vi "FilterComparison.vi"() -> ()   [LabVIEW 2019]
uses:
  <vilib>/Rock Robotics/WPI/ThirdParty/JAS_Junk/TrajLib/Trajectory_Library.lvlib
  <vilib>/Rock Robotics/WPI/ThirdParty/JAS_Junk/TrajLib/LinearFilter_MovingAvg_Execute.vi
  <vilib>/Rock Robotics/WPI/ThirdParty/JAS_Junk/TrajLib/LinearFilter_LP_BW1_Execute.vi
  <vilib>/Rock Robotics/WPI/ThirdParty/JAS_Junk/TrajLib/LinearFilter_LP_BW2_Execute.vi
  <vilib>/Rock Robotics/WPI/ThirdParty/JAS_Junk/TrajLib/LinearFilter_HP_BW1_Execute.vi
  <vilib>/Rock Robotics/WPI/ThirdParty/JAS_Junk/TrajLib/LinearFilter_HP_BW2_Execute.vi
panel:
  out "Wait Adjust":dbl format="%11.3f"
  in  "Auto / Manual":bool=TRUE
  in  "Enable\nNoise":bool=TRUE
  in  "Filter Enable":bool=TRUE
  in  "Use White Noise":bool=TRUE
  in  "Tab Control 2":T1(tab)
  out "Avg3":cluster{dbl, dbl, "Value_Output":dbl}(graph)
  out "Avg3 Out Dial":dbl(knob)=-2.895988890827539e-05 scale=-20.0..20.0
  out "Avg3 Out":dbl format="%11.3f"
  out "Med3":cluster{dbl, dbl, "Value_Output":dbl}(graph)
  out "Med3 Out":dbl format="%11.3f"
  out "Med3 Out Dial":dbl(knob)=-2.895988890827539e-05 scale=-20.0..20.0
  out "Avg7":cluster{dbl, dbl, "Value_Output":dbl}(graph)
  out "Avg7 Out":dbl format="%11.3f"
  out "Avg7 Out Dial":dbl(knob)=-2.895988890827539e-05 scale=-20.0..20.0
  out "Med7":cluster{dbl, dbl, "Value_Output":dbl}(graph)
  out "Med7 Out":dbl format="%11.3f"
  out "Med7 Out Dial":dbl(knob)=-2.895988890827539e-05 scale=-20.0..20.0
  out "LP BW 2":cluster{dbl, dbl, "Output_Value":dbl}(graph)
  out "LP BW 1 Out":dbl format="%11.3f"
  out "Low Pass 1st order Butterworth FIlter":dbl(knob)=-2.895988890827539e-05 scale=-20.0..20.0
  out "Fc 2":dbl format="%11.3f"
  out "LP BW 2":cluster{dbl, dbl, "Output_Value":dbl}(graph)
  out "LP BW 2 Out":dbl format="%11.3f"
  out "Low Pass 2nd order Butterworth Filter":dbl(knob)=-2.895988890827539e-05 scale=-20.0..20.0
  out "Fc 3":dbl format="%11.3f"
  out "HP BW 1":cluster{dbl, dbl, "Output_Value":dbl}(graph)
  out "HP BW 1":dbl format="%11.3f"
  out "High Pass 1st order Butterworth Filter":dbl(knob)=-2.895988890827539e-05 scale=-20.0..20.0
  out "HP  BW 2":cluster{dbl, dbl, "Output_Value":dbl}(graph)
  out "HP BW 2 out":dbl format="%11.3f"
  out "High Pass 2nd order Butterworth Filter":dbl(knob)=-2.895988890827539e-05 scale=-20.0..20.0
  out "Cutoff Freq\nHP BW 2":dbl format="%11.3f"
  out "Duration":dbl format="%11.3f"
  out "Late":dbl format="%11.3f"
  in  "Manual\nInput":dbl(slide) min=-12.0 max=12.0 scale=-12.0..12.0
  out "Raw Noise":dbl(knob)=-2.895988890827539e-05 scale=-20.0..20.0
  out "Raw Noise":dbl format="%11.3f"
  out "Actual Input":dbl(knob)=-2.895988890827539e-05 scale=-20.0..20.0
  out "Actual Input":dbl format="%11.3f"
  in  "Time Const (Sec)":dbl=0.08 min=0.0 step=0.001 format="%10.4f"
  out "Input":cluster{"Manual\nInput":dbl, dbl, "f":dbl}(graph)
  out "Meas Dial":dbl(knob)=-2.895988890827539e-05 scale=-20.0..20.0
  out "Measured Value":dbl format="%11.3f"
  # "Comparison of Different Filters"
  # "Loop Information"
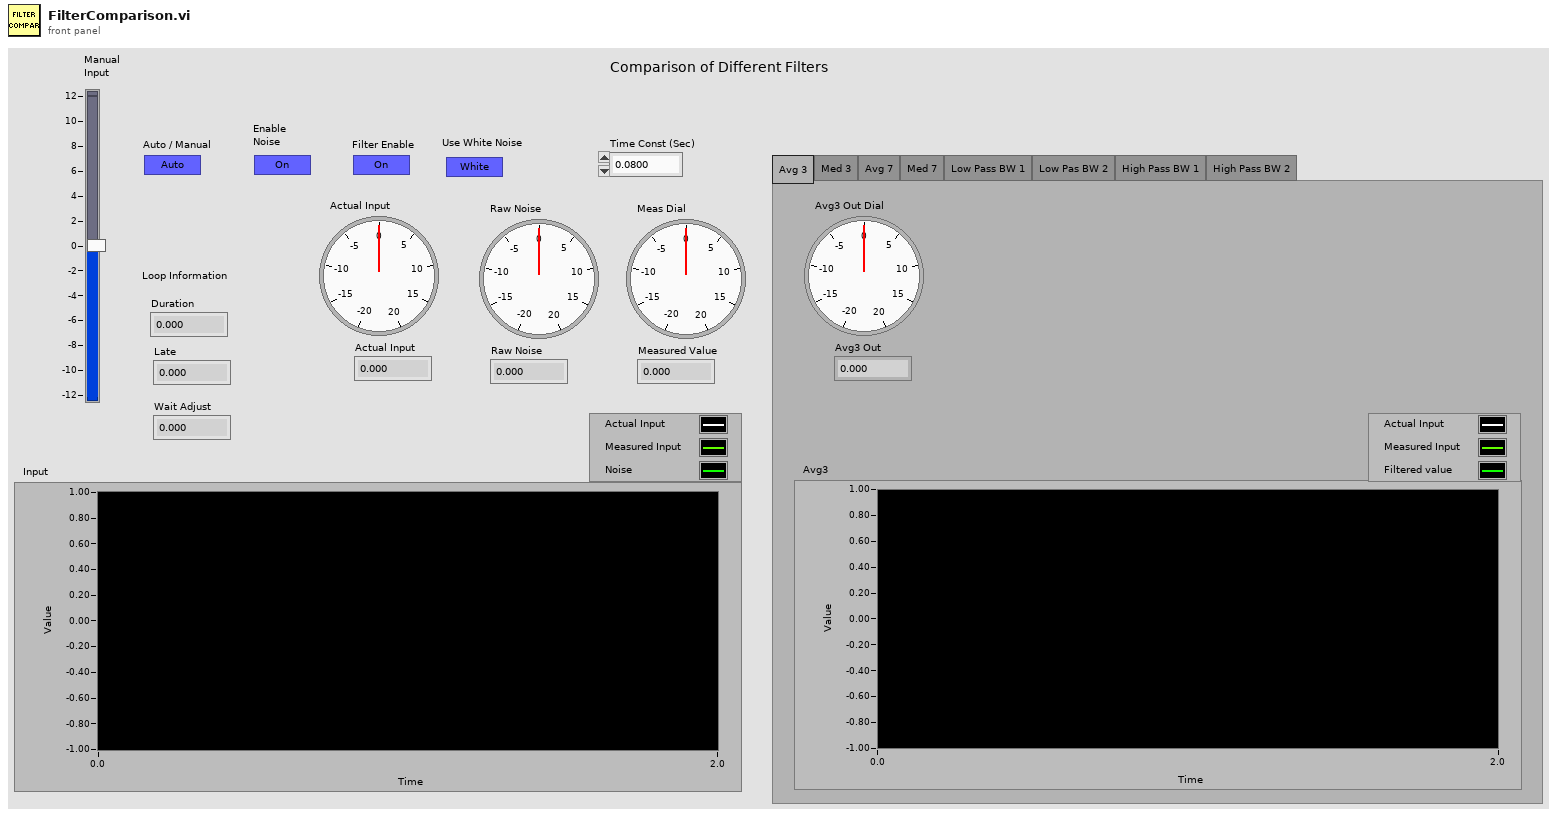
[diagram p1: front panel]
types:
  T1 = enum32{"Avg 3", "Med 3", "Avg 7", "Med 7", "Low Pass BW 1", "Low Pas BW 2", "High Pass BW 1", "High Pass BW 2"}
  T2 = cluster{"Manual\nInput":dbl, dbl, "MedianValue":dbl}
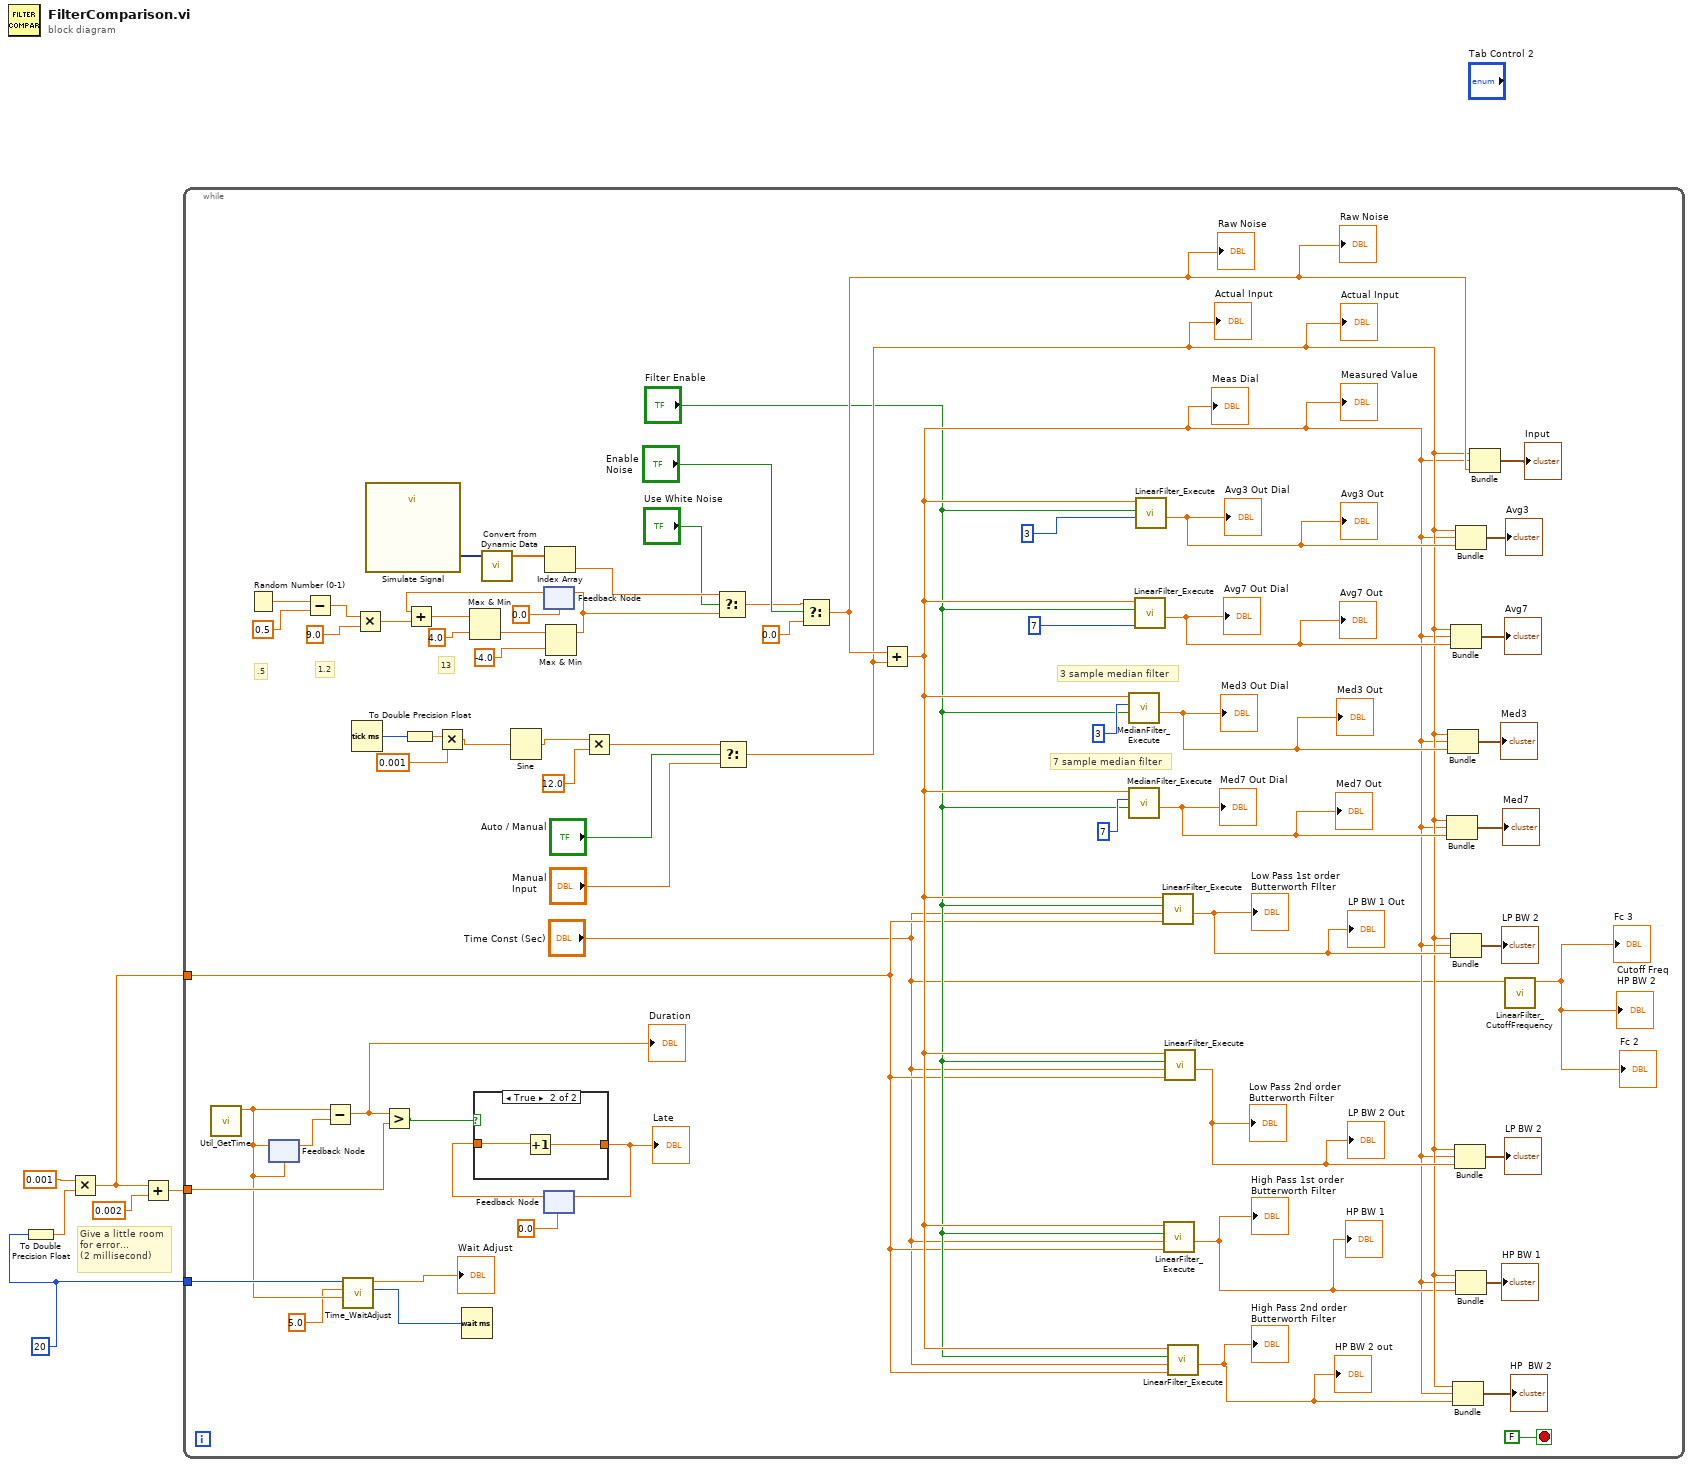
[diagram p0: block diagram]
diagram:
  w4 = u32 20 ("milliseconds to wait")
  # "Give a little room\nfor error...\n(2 millisecond)"
  n1 = To Double Precision Float(number=w4) -> (double precision float=w6:dbl)
  n2 = Multiply(x=0.001, y=w6) -> (x*y=w1:dbl)
  n3 = Add(x=w1, y=0.002) -> (x+y=w3:dbl)
  n4 = while {
    tunnel: w4 -> [w12]
    tunnel: w3 -> [w30]
    tunnel: w1 -> [w14]
    stop <- FALSE stop-if-true
    # "7 sample median filter"
    # "3 sample median filter"
    # "13"
    # "1.2"
    # ".5"
    n5 = call <vilib>:"Util_GetTime.vi"() -> ("FPGA_Time_Seconds"=w11:dbl)  [unwired: 9 in, 2 out]
    n6 = Random Number (0-1)() -> (number: 0 to 1=w70:dbl)
    n7 = feedback-in #1(w11) -> ()
    n8 = feedback #1(w11) -> (w33:dbl)
    n9 = Subtract(x=w70, y=0.5) -> (x-y=w66:dbl)
    n10 = Subtract(x=w11, y=w33) -> (x-y=w31:dbl)
    "Duration" <- w31
    n11 = call <vilib>:"Time_WaitAdjust.vi"("PassthroughTime_SEC"=w11, "MaxAdjustment_MS"=5.0 ("MaxDeviation_MS"), "DesiredLoopTime_MS"=w12) -> ("AdjustedWaitTime_MS"=w9:u32, "Offset_MS"=→"Wait Adjust":dbl)  [unwired: 7 in]
    n12 = Tick Count (ms)() -> (millisecond timer value=w59:u32)
    n13 = Multiply(x=w66, y=9.0) -> (x*y=w65:dbl)
    n14 = call "Simulate Signal"() -> ("DC with Uniform Noise"=w47:dynamicdata)  [unwired: 14 in, 1 out]
    n15 = Greater?(x=w31, y=w30) -> (0:w32:bool)
    n16 = To Double Precision Float(number=w59) -> (double precision float=w60:dbl)
    n17 = Multiply(x=w60, y=0.001) -> (x*y=w57:dbl)
    n18 = Wait (ms)(milliseconds to wait=w9) -> ()  [unwired: 1 out]
    n19 = call "Convert from Dynamic Data"("Dynamic Data Type"=w47) -> ("Array"=w46:dbl[])  [unwired: 3 in]
    n20 = Sine(x=w57) -> (sin(x)=w56:dbl)
    n21 = feedback #2(0.0) -> (w67:dbl)
    n22 = Add(x=w67, y=w65) -> (x+y=w69:dbl)
    n23 = Max & Min(x=w69, y=4.0) -> (min(x,y)=w68:dbl)  [unwired: 1 out]
    n24 = feedback #3(0.0) -> (w40:dbl)
    n25 = case shown="True" w32 {
      tunnel: [w76 w78] -> w41
      tunnel: w40 -> [w76 w77]
      frame False {
      }
      frame True {
        n26 = Increment(x=w77) -> (x+1=w78:dbl)
      }
    }
    "Late" <- w41
    n27 = feedback-in #3(w41) -> ()
    n28 = Index Array(array=w46) -> (element=w45:dbl)  [unwired: 1 in]
    n29 = Max & Min(x=w68, y=-4.0) -> (max(x,y)=w48:dbl)  [unwired: 1 out]
    n30 = feedback-in #2(w48) -> ()
    n31 = Multiply(x=w56, y=12.0) -> (x*y=w53:dbl)
    n32 = Select(t=w45, s="Use White Noise", f=w48) -> (s? t:f=w49:dbl)
    n33 = Select(t=w53, s="Auto / Manual", f="Manual\nInput") -> (s? t:f=w21:dbl)
    "Actual Input" <- w21
    "Actual Input" <- w21
    n34 = Select(t=w49, s="Enable\nNoise", f=0.0) -> (s? t:f=w43:dbl)
    "Raw Noise" <- w43
    "Raw Noise" <- w43
    n35 = Add(x=w43, y=w21) -> (x+y=w16:dbl)
    "Measured Value" <- w16
    "Meas Dial" <- w16
    n36 = call <vilib>:"MedianFilter_Execute.vi"("Enable"="Filter Enable", "Samples"=3, "Input Value"=w16) -> ("MedianValue"=w26:dbl)  [unwired: 7 in, 1 out]
    "Med3 Out" <- w26
    "Med3 Out Dial" <- w26
    n37 = call <vilib>:"MedianFilter_Execute.vi"("Enable"="Filter Enable", "Samples"=7, "Input Value"=w16) -> ("MedianValue"=w28:dbl)  [unwired: 7 in, 1 out]
    "Med7 Out" <- w28
    "Med7 Out Dial" <- w28
    n38 = call-poly <vilib>:"LinearFilter_Execute.vi"("Samples"=7, "Enable"="Filter Enable", "Input"=w16) -> ("Output"=w35:dbl)  [unwired: 8 in]
    "Avg7 Out" <- w35
    "Avg7 Out Dial" <- w35
    n39 = call-poly <vilib>:"LinearFilter_Execute.vi"("Samples"=3, "Enable"="Filter Enable", "Input"=w16) -> ("Output"=w36:dbl)  [unwired: 8 in]
    "Avg3 Out" <- w36
    "Avg3 Out Dial" <- w36
    n40 = call-poly <vilib>:"LinearFilter_Execute.vi"("SamplePeriod"=w14, "TimeConstant"="Time Const (Sec)", "Enable"="Filter Enable", "Input"=w16) -> ("Output"=w29:dbl)  [unwired: 7 in]
    "LP BW 1 Out" <- w29
    "Low Pass 1st order Butterworth FIlter" <- w29
    n41 = call-poly <vilib>:"LinearFilter_Execute.vi"("SamplePeriod"=w14, "TimeConstant"="Time Const (Sec)", "Enable"="Filter Enable", "Input"=w16) -> ("Output"=w17:dbl)  [unwired: 7 in]
    "High Pass 1st order Butterworth Filter" <- w17
    "HP BW 1" <- w17
    n42 = call-poly <vilib>:"LinearFilter_Execute.vi"("SamplePeriod"=w14, "TimeConstant"="Time Const (Sec)", "Enable"="Filter Enable", "Input"=w16) -> ("Output"=w22:dbl)  [unwired: 7 in]
    "LP BW 2 Out" <- w22
    "Low Pass 2nd order Butterworth Filter" <- w22
    n43 = call-poly <vilib>:"LinearFilter_Execute.vi"("SamplePeriod"=w14, "TimeConstant"="Time Const (Sec)", "Enable"="Filter Enable", "Input"=w16) -> ("Output"=w18:dbl)  [unwired: 7 in]
    "HP BW 2 out" <- w18
    "High Pass 2nd order Butterworth Filter" <- w18
    n44 = Bundle("Manual\nInput"=w21, w16, "MedianValue"=w28) -> (→"Med7":T2)  [unwired: 1 in]
    n45 = Bundle("Manual\nInput"=w21, w16, "MedianValue"=w26) -> (→"Med3":T2)  [unwired: 1 in]
    n46 = Bundle("Manual\nInput"=w21, w16, "Output"=w35) -> (→"Avg7":cluster{"Manual\nInput":dbl, dbl, "Output":dbl})  [unwired: 1 in]
    n47 = Bundle("Manual\nInput"=w21, w16, "Output"=w29) -> (→"LP BW 2":cluster{"Manual\nInput":dbl, dbl, "Output":dbl})  [unwired: 1 in]
    n48 = Bundle("Manual\nInput"=w21, w16, "Output"=w18) -> (→"HP  BW 2":cluster{"Manual\nInput":dbl, dbl, "Output":dbl})  [unwired: 1 in]
    n49 = Bundle("Manual\nInput"=w21, w16, "Output"=w22) -> (→"LP BW 2":cluster{"Manual\nInput":dbl, dbl, "Output":dbl})  [unwired: 1 in]
    n50 = Bundle("Manual\nInput"=w21, w16, "Output"=w36) -> (→"Avg3":cluster{"Manual\nInput":dbl, dbl, "Output":dbl})  [unwired: 1 in]
    n51 = Bundle("Manual\nInput"=w21, w16, "Output"=w17) -> (→"HP BW 1":cluster{"Manual\nInput":dbl, dbl, "Output":dbl})  [unwired: 1 in]
    n52 = Bundle("Manual\nInput"=w21, w16, "f"=w43) -> (→"Input":cluster{"Manual\nInput":dbl, dbl, "f":dbl})  [unwired: 1 in]
    n53 = call <vilib>:"LinearFilter_CutoffFrequency.vi"("TimeConstant"="Time Const (Sec)") -> ("Cutoff Freq"=→"Cutoff Freq\nHP BW 2" →"Fc 2" →"Fc 3":dbl)  [unwired: 10 in]
  }
